vi "Update_MemBank.vi"(8 "error in":errorcluster, 10 "NNPC_MemBank_and_Params":T1={"MemBank_Data"={"MemBank"=variant, "MemBank Norm"=variant}, "PreProc_Options"={"DS_Name"="", "Input_Dims"={"C"=-1, "H"=-1, "W"=-1}, "Cropping"={"Left"=0.0, "Top"=0.0, "Right"=1.0, "Bottom"=1.0}, "Interpolation Type"=1, "MultiStage_ReSample?"=FALSE, "Dataset_Stats"={"means"={"R"=0.5385, "G"=0.5348, "B"=0.551}, "stds"={"R"=0.3673, "G"=0.3673, "B"=0.3505}}}, "Evaluation_Results"={"Threshold(Image)"=0.0, "Threshold(Pixel)"=0.0, "Pixel_Range"={"Min"=0.0, "Max"=0.0}}, "MemBank on GPU?"=FALSE} {"PreProc_Options"."Dataset_Stats"."stds"."R" format="%#_3g"; "PreProc_Options"."Dataset_Stats"."stds"."G" format="%#_3g"; "PreProc_Options"."Dataset_Stats"."stds"."B" format="%#_3g"; "PreProc_Options"."Dataset_Stats"."means"."R" format="%#_3g"; "PreProc_Options"."Dataset_Stats"."means"."G" format="%#_3g"; "PreProc_Options"."Dataset_Stats"."means"."B" format="%#_3g"; "PreProc_Options"."Interpolation Type" items=["Zero Order", "Bi-Linear", "Quadratic", "Cubic Spline"]; "Evaluation_Results"."Pixel_Range"."Min" format="%#_5g"}, 11 "NNPC_out in":T9 {"NN"."LR_Update_Policy"."WarmUp_Ratio" min=1; "NN"."LR_Update_Policy"."WarmUp_Iter" min=1; "NN"."LR_Update_Policy"."LR0" format="%.7f"}) -> (0 "error out":errorcluster, 3 "NNPC_out out":T9 {"NN"."LR_Update_Policy"."WarmUp_Ratio" min=1; "NN"."LR_Update_Policy"."WarmUp_Iter" min=1; "NN"."LR_Update_Policy"."LR0" format="%.7f"})   [LabVIEW 2020]
uses:
  <vilib>/Ngene/DeepLTK Anomaly Detection Addon/Toolkit/API/Controls/NNPC_Instance.ctl
  <vilib>/Ngene/Deep Learning Toolkit/Toolkit/NN_Network/Controls/NN.ctl
  <vilib>/Ngene/Deep Learning Toolkit/Toolkit/NN_Layers/Controls/NN_Layer_ref.ctl
  <vilib>/Ngene/Deep Learning Toolkit/Toolkit/NN_Network/Controls/NN_In_Out_Dim-ty.ctl
  <vilib>/Ngene/Deep Learning Toolkit/Toolkit/NN_Data/API/NN_Dims(C,H,W).ctl
  <vilib>/Ngene/Deep Learning Toolkit/Toolkit/NN_Train/Controls/NN_Train_Params.ctl
  <vilib>/Ngene/Deep Learning Toolkit/Toolkit/NN_Train/Controls/NN_Train_Optimizer.ctl
  <vilib>/Ngene/Deep Learning Toolkit/Toolkit/NN_Train/Controls/NN_Train_Data_Sampling.ctl
  <vilib>/Ngene/Deep Learning Toolkit/Toolkit/NN_Train/Controls/NN_LR_Policy_Cfg.ctl
  <vilib>/Ngene/Deep Learning Toolkit/Toolkit/NN_Train/Controls/NN_LR_Policy_Type.ctl
  <vilib>/Ngene/Deep Learning Toolkit/Toolkit/NN_Train/Controls/NN_Train_Session_Data.ctl
  <vilib>/Ngene/Deep Learning Toolkit/Toolkit/NN_Data/Controls/NN_Ground_truth.ctl
  <vilib>/Ngene/Deep Learning Toolkit/Toolkit/NNg/cuda/Controls/nng_cuda_handles.ctl
  <vilib>/Ngene/Deep Learning Toolkit/Toolkit/NN_Network/Controls/NN_Device.ctl
  <vilib>/Ngene/Deep Learning Toolkit/Toolkit/NN_Train/Controls/NN_Loss_Type.ctl
  <vilib>/Ngene/Deep Learning Toolkit/Toolkit/NNg/Network/WS/Controls/NNG_WS.ctl
  <vilib>/Ngene/Deep Learning Toolkit/Toolkit/NNg/Network/WS/Controls/NNg_WS_Mem_DVR.ctl
  <vilib>/Ngene/Deep Learning Toolkit/Toolkit/NNg/cuda/Controls/cuda_Mem_desc.ctl
  <vilib>/Ngene/DeepLTK Anomaly Detection Addon/Toolkit/API/Controls/MemBank_and_Norm_Variants.ctl
  Controls/NNPC_MemBank_and_Params.ctl
  <vilib>/Ngene/DeepLTK Anomaly Detection Addon/Toolkit/API/Controls/NNPC_PreProcessing_Options.ctl
  <vilib>/Ngene/DeepLTK Anomaly Detection Addon/Toolkit/API/Controls/Crop_CFG.ctl
  <vilib>/Ngene/DeepLTK Anomaly Detection Addon/Toolkit/API/Controls/NNPC_DS_Stats.ctl
  <vilib>/Ngene/DeepLTK Anomaly Detection Addon/Toolkit/API/Controls/Image_Stats_RGB.ctl
  <vilib>/Ngene/DeepLTK Anomaly Detection Addon/Toolkit/API/Controls/NNPC_Evaluation_Results.ctl
  <vilib>/Ngene/CuLab - GPU Accelerated Toolkit/Toolkit/Low_Level/Tensor_Classes/T_Children/T2D/T2D_Children/T2D_SGL/Push.vi
  <vilib>/Ngene/CuLab - GPU Accelerated Toolkit/Toolkit/Low_Level/Tensor_Classes/T_Children/T1D/T1D_Children/T1D_SGL/Push.vi
  <vilib>/Ngene/Deep Learning Toolkit/Toolkit/Deep_Learning_Toolkit_by_Ngene.lvlib
  <vilib>/Ngene/CuLab - GPU Accelerated Toolkit/Toolkit/CuLab.lvlib
  <vilib>/Ngene/DeepLTK Anomaly Detection Addon/Toolkit/DeepLTK_Anomaly_Detection_Addon.lvlib
  <vilib>/Ngene/CuLab - GPU Accelerated Toolkit/Toolkit/Low_Level/Tensor_Classes/T_Children/T1D/T1D_Children/T1D_SGL/T1D_SGL.lvclass
  <vilib>/Ngene/CuLab - GPU Accelerated Toolkit/Toolkit/Low_Level/Tensor_Classes/T_Children/T2D/T2D_Children/T2D_SGL/T2D_SGL.lvclass
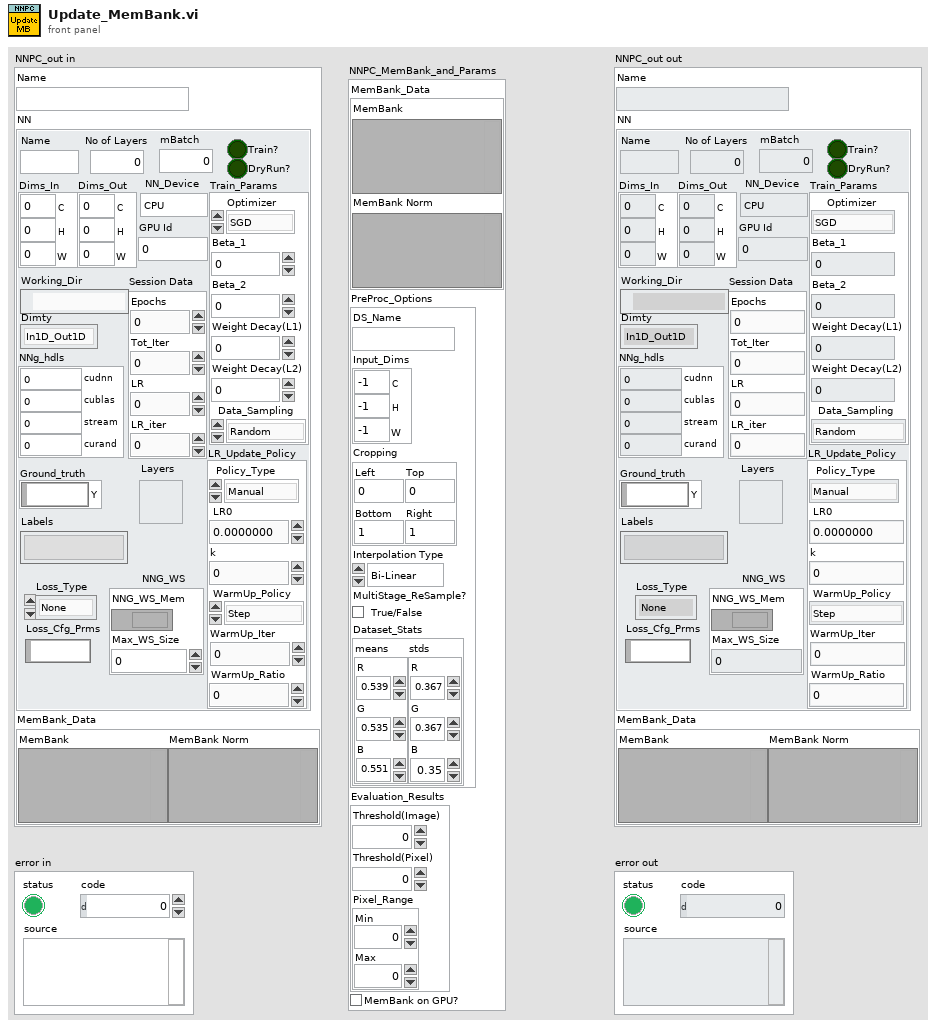
[diagram p1: front panel]
types:
  T1 = typedef "NNPC_MemBank_and_Params.ctl" = cluster{"MemBank_Data":T2, "PreProc_Options":T3, "Evaluation_Results":T8, "MemBank on GPU?":bool}
  T2 = typedef "DeepLTK_Anomaly_Detection_Addon.lvlib/MemBank_and_Norm_Variants.ctl" = cluster{"MemBank":variant, "MemBank Norm":variant}
  T3 = typedef "DeepLTK_Anomaly_Detection_Addon.lvlib/NNPC_PreProcessing_Options.ctl" = cluster{"DS_Name":string, "Input_Dims":T4, "Cropping":T5, "Interpolation Type":u32, "MultiStage_ReSample?":bool, "Dataset_Stats":T6}
  T4 = typedef "Deep_Learning_Toolkit_by_Ngene.lvlib/NN_Dims(C,H,W).ctl" = cluster{"C":i32, "H":i32, "W":i32}
  T5 = typedef "DeepLTK_Anomaly_Detection_Addon.lvlib/Crop_CFG.ctl" = cluster{"Left":sgl, "Top":sgl, "Right":sgl, "Bottom":sgl}
  T6 = typedef "DeepLTK_Anomaly_Detection_Addon.lvlib/NNPC_DS_Stats.ctl" = cluster{"means":T7, "stds":T7}
  T7 = typedef "DeepLTK_Anomaly_Detection_Addon.lvlib/Image_Stats_RGB.ctl" = cluster{"R":sgl, "G":sgl, "B":sgl}
  T8 = typedef "DeepLTK_Anomaly_Detection_Addon.lvlib/NNPC_Evaluation_Results.ctl" = cluster{"Threshold(Image)":sgl, "Threshold(Pixel)":sgl, "Pixel_Range":cluster{"Min":sgl, "Max":sgl}}
  T9 = typedef "DeepLTK_Anomaly_Detection_Addon.lvlib/NNPC_Instance.ctl" = cluster{"Name":string, "NN":T10, "MemBank_Data":T2}
  T10 = typedef "Deep_Learning_Toolkit_by_Ngene.lvlib/NN.ctl" = cluster{"Name":string, "No of Layers":i32, "mBatch":i32, "Layers":T11[], "Dimty":T12, "Dims_In":T4, "Dims_Out":T4, "Working_Dir":path, "Train?":bool, "Train_Params":T13, "LR_Update_Policy":T16, "Session Data":T18, "Ground_truth":T19, "NNg_hdls":T20, "NN_Device":T21, "GPU Id":i32, "Labels":string[], "Loss_Type":T22, "Loss_Cfg_Prms":variant, "NNG_WS":T23, "DryRun?":bool}
  T11 = typedef "Deep_Learning_Toolkit_by_Ngene.lvlib/NN_Layer_ref.ctl" = refnum<file>
  T12 = typedef "Deep_Learning_Toolkit_by_Ngene.lvlib/NN_In_Out_Dim-ty.ctl" = enum8{"In1D_Out1D", "In3D_Out1D", "In3D_Out3D", "In3D_OutBBox"}
  T13 = typedef "Deep_Learning_Toolkit_by_Ngene.lvlib/NN_Train_Params.ctl" = cluster{"Optimizer":T14, "Beta_1":sgl, "Beta_2":sgl, "Weight Decay(L1)":sgl, "Weight Decay(L2)":sgl, "Data_Sampling":T15}
  T14 = typedef "Deep_Learning_Toolkit_by_Ngene.lvlib/NN_Train_Optimizer.ctl" = enum16{"SGD", "Adam", "Adagrad", "Adadelta", "RMSProp", "Nesterov"}
  T15 = typedef "Deep_Learning_Toolkit_by_Ngene.lvlib/NN_Train_Data_Sampling.ctl" = enum16{"Random", "Sequential"}
  T16 = typedef "Deep_Learning_Toolkit_by_Ngene.lvlib/NN_LR_Policy_Cfg.ctl" = cluster{"Policy_Type":T17, "LR0":dbl, "k":sgl, "WarmUp_Policy":enum16{"Step", "Ramp"}, "WarmUp_Iter":i32, "WarmUp_Ratio":sgl}
  T17 = typedef "Deep_Learning_Toolkit_by_Ngene.lvlib/NN_LR_Policy_Type.ctl" = enum16{"Manual", "Step", "Exp", "1/t"}
  T18 = typedef "Deep_Learning_Toolkit_by_Ngene.lvlib/NN_Train_Session_Data.ctl" = cluster{"Epochs":sgl, "Tot_Iter":i32, "LR":sgl, "LR_iter":i32}
  T19 = typedef "Deep_Learning_Toolkit_by_Ngene.lvlib/NN_Ground_truth.ctl" = cluster{"Y":variant}
  T20 = typedef "Deep_Learning_Toolkit_by_Ngene.lvlib/nng_cuda_handles.ctl" = cluster{"cudnn":u64, "cublas":u64, "stream":u64, "curand":u64}
  T21 = typedef "Deep_Learning_Toolkit_by_Ngene.lvlib/NN_Device.ctl" = enum16{"CPU", "GPU"}
  T22 = typedef "Deep_Learning_Toolkit_by_Ngene.lvlib/NN_Loss_Type.ctl" = enum16{"None", "MSE", "CrossEntropy", "YOLO_v2", "YOLO_v4"}
  T23 = typedef "Deep_Learning_Toolkit_by_Ngene.lvlib/NNG_WS.ctl" = cluster{"NNG_WS_Mem":T24, "Max_WS_Size":i64}
  T24 = typedef "Deep_Learning_Toolkit_by_Ngene.lvlib/NNg_WS_Mem_DVR.ctl" = refnum<data-value>
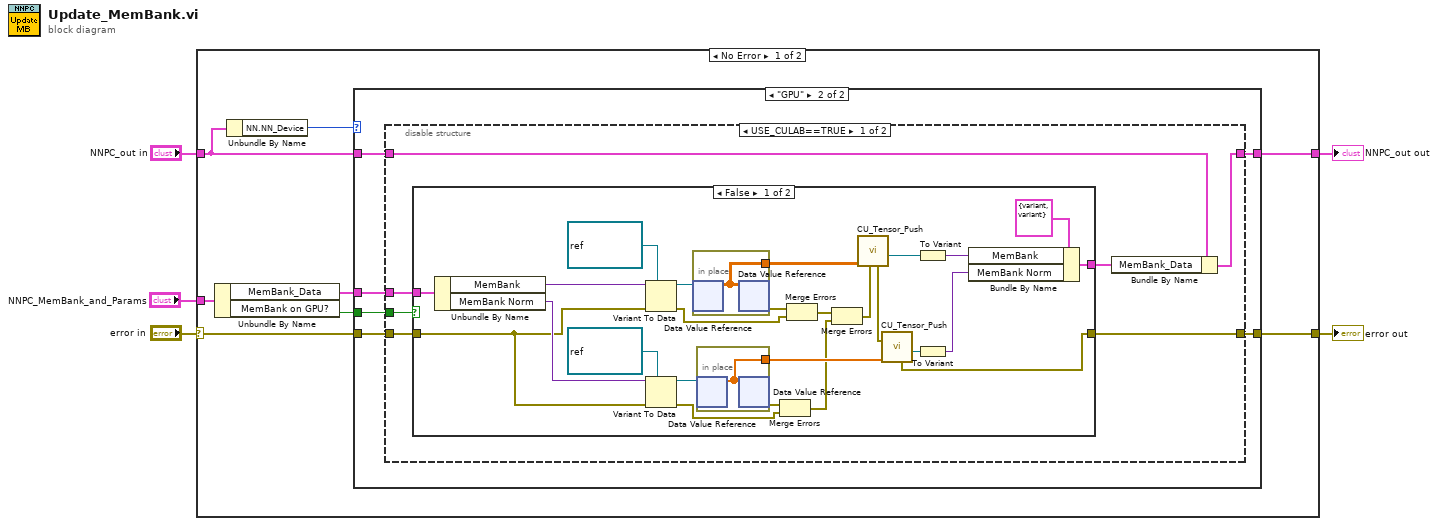
[diagram p0: block diagram]
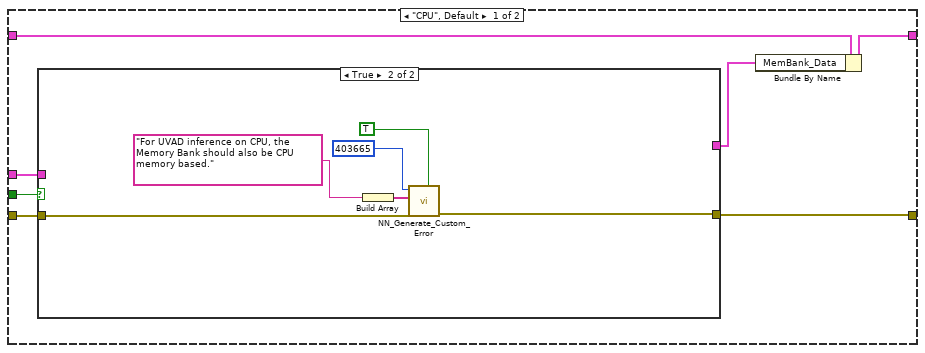
[diagram p2: hidden frame]
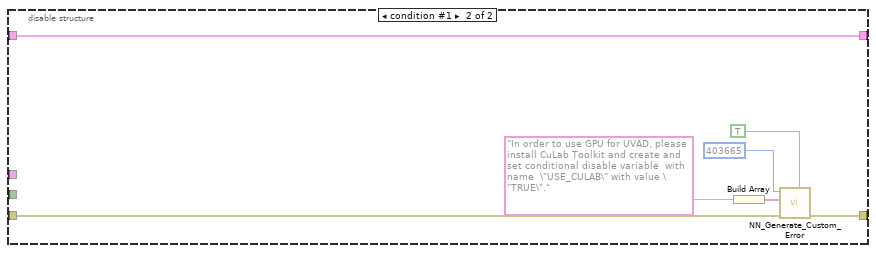
[diagram p5: hidden frame]
diagram:
  n1 = case shown="No Error" "error in" {
    selector: "error in" -> [w9 w78]
    tunnel: "NNPC_MemBank_and_Params" -> [w13 _]
    tunnel: [w12 w79] -> w5
    tunnel: "NNPC_out in" -> [w11 w79]
    tunnel: [w8 w78] -> w2
    frame No Error {
      n2 = Unbundle By Name(w13) -> ("MemBank_Data"=w7:T2, "MemBank on GPU?"=w6:bool)
      n3 = Unbundle By Name(w11) -> ("NN.NN_Device"=w10:T21)
      n4 = case shown="\"GPU\"" w10 {
        tunnel: w7 -> [w18 w34]
        tunnel: [w19 w33] -> w12
        tunnel: w11 -> [w20 w32]
        tunnel: w9 -> [w16 w31]
        tunnel: [w15 w30] -> w8
        tunnel: w6 -> [w17 w29]
        frame "CPU", Default {
          n5 = case shown="True" w17 {
            tunnel: [w22 _] -> w14
            tunnel: w18 -> [w22 _]
            tunnel: w16 -> [w21 w24]
            tunnel: [w21 w23] -> w15
            frame False {
            }
            frame True {
              n6 = Build Array("For UVAD inference on CPU, the Memory Bank should also be CPU memory based." ("Message")) -> (w28:string[])
              n7 = call <vilib>:"NN_Generate_Custom_Error.vi"("show call chain? (TRUE)"=TRUE ("show call chain? (False)"), "error in (no error)"=w24, "Message"=w28, "Error_code"=403665) -> ("error out"=w23:errorcluster)  [unwired: 7 in]
            }
          }
          n8 = Bundle By Name(cluster=w20, "MemBank_Data"=w14) -> (w19:T9)
        }
        frame "GPU" {
          n9 = disable-structure shown="USE_CULAB==TRUE" {
            disable-tunnel: w34 -> [w37 _]
            disable-tunnel: [w41 w73] -> w33
            disable-tunnel: w32 -> [w40 w73]
            disable-tunnel: w31 -> [w36 w72]
            disable-tunnel: [w35 w71] -> w30
            disable-tunnel: w29 -> [w39 _]
            frame condition #0 (active) {
              n10 = case shown="False" w39 {
                tunnel: [w43 w70] -> w38
                tunnel: w37 -> [w46 w70]
                tunnel: w36 -> [w45 w69]
                tunnel: [w42 w69] -> w35
                frame False {
                  n11 = Unbundle By Name(w46) -> ("MemBank"=w65:variant, "MemBank Norm"=w60:variant)
                  n12 = Variant To Data(error in=w45, type=refnum<data-value> refnum ("MemBank DVR"), Variant=w65) -> (data=w52:refnum<data-value>, error out=w48:errorcluster)
                  n13 = Variant To Data(error in=w45, type=refnum<data-value> refnum ("data value reference"), Variant=w60) -> (data=w47:refnum<data-value>, error out=w50:errorcluster)
                  n14 = in-place {
                    in-place-border: [w68] -> w64
                    n15 = in-place-dvr #1(w52) -> (w68:sgl[][])  [unwired: 1 out]
                    n16 = in-place-dvr #1(w68) -> (w56:errorcluster)  [unwired: 1 out]
                  }
                  n17 = in-place {
                    in-place-border: [w67] -> w58
                    n18 = in-place-dvr #2(w47) -> (w67:sgl[])  [unwired: 1 out]
                    n19 = in-place-dvr #2(w67) -> (w55:errorcluster)  [unwired: 1 out]
                  }
                  n20 = Merge Errors(w55, w50) -> (w51:errorcluster)
                  n21 = Merge Errors(w56, w48) -> (w49:errorcluster)
                  n22 = Merge Errors(w49, w51) -> (w57:errorcluster)
                  n23 = call-poly <vilib>:"CU_Tensor_Push.vi"("error in (no error)"=w57, "CPU_Data_2D_SGL"=w64) -> ("T2D_SGL out"=w63:refnum<class "T2D_SGL.lvclass">, "error out"=w54:errorcluster)  [unwired: 7 in, 1 out]
                  n24 = call-poly <vilib>:"CU_Tensor_Push.vi"("error in (no error)"=w54, "CPU_Data_1D_SGL"=w58) -> ("T1D_SGL out"=w59:refnum<class "T1D_SGL.lvclass">, "error out"=w42:errorcluster)  [unwired: 7 in, 1 out]
                  n25 = To Variant(anything=w63) -> (Variant=w62:variant)
                  n26 = To Variant(anything=w59) -> (Variant=w53:variant)
                  n27 = Bundle By Name(cluster=T2 {"MemBank"=variant, "MemBank Norm"=variant} ("MemBank_Data"), "MemBank"=w62, "MemBank Norm"=w53) -> (w43:T2)
                }
                frame True {
                }
              }
              n28 = Bundle By Name(cluster=w40, "MemBank_Data"=w38) -> (w41:T9)
            }
            frame condition #1 {
              n29 = Build Array("In order to use GPU for UVAD, please install CuLab Toolkit and create and set conditional disable variable  with name  \"USE_CULAB\" with value \"TRUE\"." ("Message")) -> (w77:string[])
              n30 = call <vilib>:"NN_Generate_Custom_Error.vi"("show call chain? (TRUE)"=TRUE ("show call chain? (False)"), "error in (no error)"=w72, "Message"=w77, "Error_code"=403665) -> ("error out"=w71:errorcluster)  [unwired: 7 in]
            }
          }
        }
      }
    }
    frame Error {
    }
  }
  "NNPC_out out" <- w5
  "error out" <- w2
